vi "Test Existing Received File is Deleted if Test Passes.vi"(11 "Test Case In":refnum<class "Basic Mechanics Tests.lvclass">) -> (0 "error out":errorcluster, 3 "Test Case Out":refnum<class "Basic Mechanics Tests.lvclass">)   [LabVIEW 2020, in "Basic Mechanics Tests.lvclass"]
uses:
  Basic Mechanics Tests.lvclass
  C:/Program Files/National Instruments/LabVIEW 2026/vi.lib/Astemes/LUnit/Test Case.lvclass
  Source/Approval Tests/Options/Options.lvclass
  Source/Approval Tests/Report Nothing/Report Nothing.lvclass
  C:/Users/SAS/Desktop/ApprovalTests.LabVIEW/Source/Approval Tests/Reporter/Reporter.lvclass
  Source/Approval Tests/Options/Options.lvclass/Options.ctl
  Source/Approval Tests/Naming Data/Naming Data.lvclass/Naming Data.ctl
  <vilib>/Astemes/LUnit/Test Case.lvclass/Test Case.ctl
  4be351cf-9afa-44a9-9686-c31d6937e1da.vi
  fbf3a6f1-25d3-4b1a-9ed1-fe282719be7b.vi
  Source/Approval Tests/Options/Write Reporter.vi
  Source/Approval Tests/Verify Core.vi
  4be351cf-9afa-44a9-9686-c31d6937e1da.vi/93c5622b-9fb7-41e0-8c76-3fde37e94e34.vi
  Source/Approval Tests/Options/Update Test Name if Not Defined.vi
  Source/Approval Tests/Options/Read Scrubber.vi
  <vilib>/Astemes/LUnit/Core/LUnit Test Case/Private/Append Fail Result.vi
  <vilib>/Astemes/LUnit/Core/LUnit Test Case/Private/Append Pass Result.vi
  fbf3a6f1-25d3-4b1a-9ed1-fe282719be7b.vi/9c5d11cd-9439-4240-a1ee-d9baace9c924.vi
  Source/Approval Tests/Options/Read Namer.vi
  Source/Approval Tests/Options/Read Naming Data.vi
  Source/Approval Tests/Options/Read Reporter.vi
  Source/Approval Tests/Options/Read Text Comparator.vi
  4be351cf-9afa-44a9-9686-c31d6937e1da.vi/93c5622b-9fb7-41e0-8c76-3fde37e94e34.vi/04cb982b-2eda-40d0-8d7e-90f8e0b569b2.vi
  Source/Approval Tests/Naming Data/Read Test VI Name.vi
  Source/Approval Tests/Naming Data/Write Test VI Name.vi
  <vilib>/Astemes/LUnit/Core/LUnit Test Case/Private/Run In UI.vi
  Source/Approval Tests/Options/Add Label to Namer.vi
  Source/Approval Tests/conv EOL.vi
  Source/Approval Tests/Reporter/Report.vi
  Source/Approval Tests/Scrubber/Scrubber.lvclass
  Source/Approval Tests/Namer/Namer.lvclass
  Source/Approval Tests/Naming Data/Naming Data.lvclass
  Source/Approval Tests/Reporter/Reporter.lvclass
  Source/Approval Tests/Text Comparator/Text Comparator.lvclass
  <vilib>/Astemes/LUnit/Test Case.lvclass
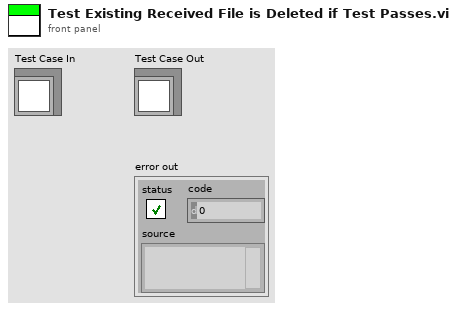
[diagram p1: front panel]
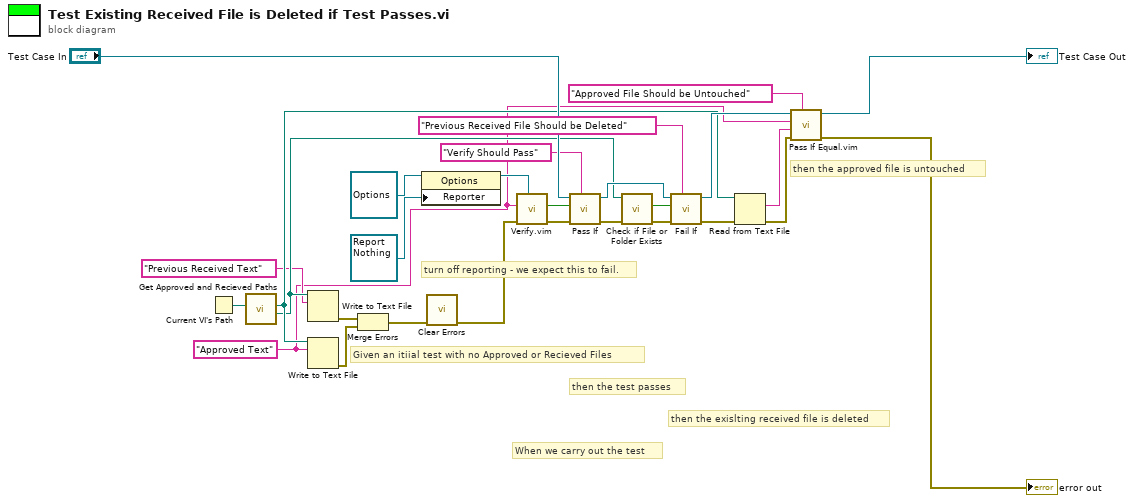
[diagram p0: block diagram]
diagram:
  w4 = "Approved Text"
  # "then the approved file is untouched"
  # "then the exislting received file is deleted"
  # "then the test passes"
  # "When we carry out the test"
  # "Given an itiial test with no Approved or Recieved Files"
  # "turn off reporting - we expect this to fail."
  n1 = Current VI's Path() -> (path=w9:path)
  n2 = call "Get Approved and Recieved Paths.vi"("This VI"=w9) -> ("Recieved"=w6:path, "Approved Path"=w7:path)  [unwired: 9 in]
  n3 = Write to Text File(file (use dialog)=w6, text="Previous Received Text") -> (error out=w20:errorcluster)  [unwired: 2 in, 2 out]
  n4 = Write to Text File(file (use dialog)=w7, text=w4) -> (error out=w21:errorcluster)  [unwired: 2 in, 2 out]
  n5 = Merge Errors(w20, w21) -> (w24:errorcluster)
  n6 = property on="Property Node" class="Options"(reference=refnum<class "Options.lvclass"> refnum ("Options"), "Reporter"=refnum<class "Report Nothing.lvclass"> refnum ("Approval Tests.lvlib:Report Nothing")) -> (reference out=w16:refnum<class "Options.lvclass">)  [unwired: 1 in, 1 out]
  n7 = call <vilib>:"Clear Errors.vi"("error in (no error)"=w24) -> ("error out"=w19:errorcluster)  [unwired: 5 in, 1 out]
  n8 = call "Verify.vim"("Options"=w16, "error in"=w19, "Anything"=w4) -> ("error out"=w25:errorcluster, "Passed?"=w14:bool)  [unwired: 6 in, 1 out]
  n9 = call <vilib>:"Pass If.vi"("Description"="Verify Should Pass", "error in (no error)"=w25, "Pass?"=w14, "LUnit Test Case In"="Test Case In") -> ("error out"=w23:errorcluster, "LUnit Test Case Out"=w13:refnum<class "Basic Mechanics Tests.lvclass">)  [unwired: 6 in]
  n10 = call <vilib>:"Check if File or Folder Exists.vi"("error in (no error)"=w23, "path"=w6) -> ("error out"=w22:errorcluster, "file or folder exists?"=w8:bool)  [unwired: 7 in, 1 out]
  n11 = call <vilib>:"Fail If.vi"("Description"="Previous Received File Should be Deleted", "error in (no error)"=w22, "Fail?"=w8, "LUnit Test Case In"=w13) -> ("error out"=w26:errorcluster, "LUnit Test Case Out"=w12:refnum<class "Basic Mechanics Tests.lvclass">)  [unwired: 6 in]
  n12 = Read from Text File(file (use dialog)=w7, error in=w26) -> (text=w10:string, error out=w27:errorcluster)  [unwired: 2 in, 2 out]
  n13 = call "Pass If Equal.vim"("Description"="Approved File Should be Untouched", "error in (no error)"=w27, "Actual"=w10, "Expected"=w4, "LUnit Test Case In"=w12) -> ("error out"=→"error out":errorcluster, "LUnit Test Case Out"=→"Test Case Out":refnum<class "Basic Mechanics Tests.lvclass">)  [unwired: 5 in]
